vi "Read CSV File.vi"(10 "文件参数":T1={"时间列"=1, "名称行"=1, "单位行"=2, "数据首行"=3, "数据首列"=2, "分隔符"=enum."逗号"}, 11 "Path":path=path "D:/同步空间/曲线生成/原始曲线/3、增达--Data.xls") -> (2 "Data Series":T2[](array[typedef]))   [LabVIEW 2020, in "Data Viewer.lvlib"]
uses:
  Data Viewer.lvlib
  Data Serie--cluster.ctl
  File Type--enum.ctl
  <vilib>/Utility/file.llb/Read Delimited Spreadsheet (string).vi
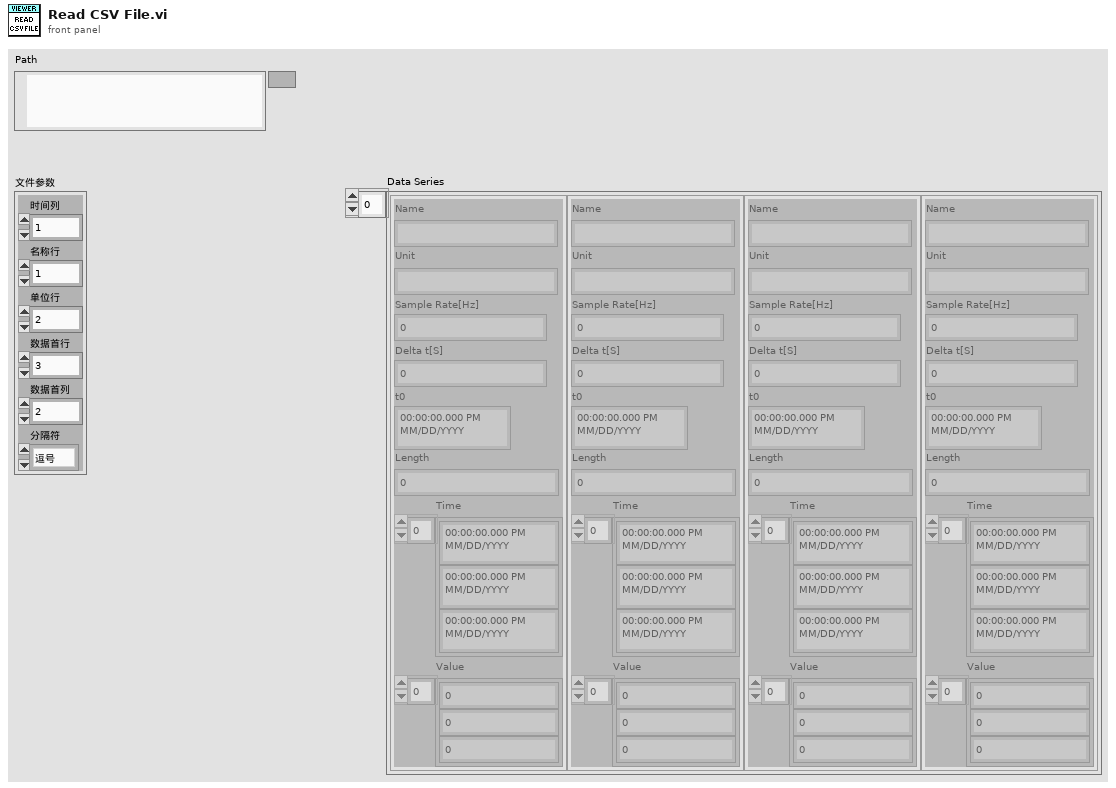
[diagram p1: front panel]
types:
  T1 = cluster{"时间列":i32, "名称行":i32, "单位行":i32, "数据首行":i32, "数据首列":i32, "分隔符":enum16{"逗号", "制表符"}}
  T2 = typedef "Data Viewer.lvlib/Data Serie--cluster.ctl" = cluster{"Name":string, "Unit":string, "Sample Rate[Hz]":dbl, "Delta t[S]":dbl, "t0":timestamp, "Length":i32, "Time":timestamp[], "Value":dbl[]}
  T3 = typedef "Data Viewer.lvlib/File Type--enum.ctl" = enum16{"伟思环境箱", "增达环境箱", "广五所环境箱", "无纸记录仪", "帕捷SA00339", "记录仪840", "记录仪8400", "记录仪MR888", "*.csv"}
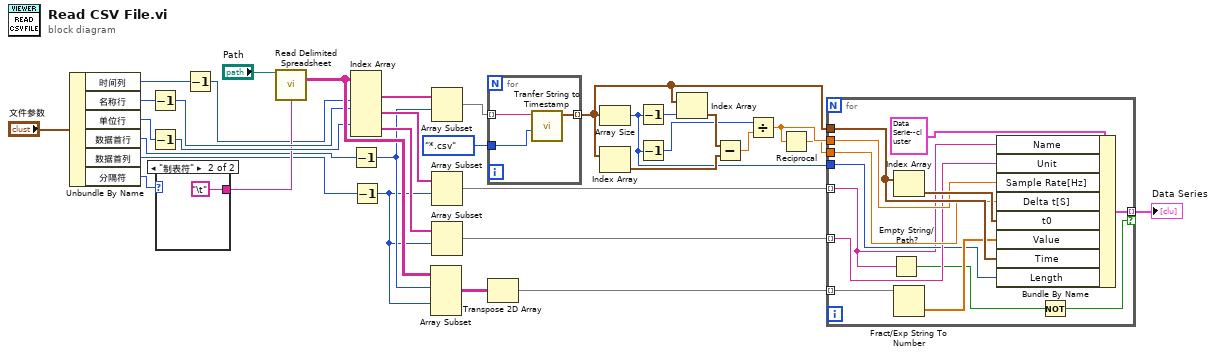
[diagram p0: block diagram]
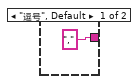
[diagram p2: hidden frame]
diagram:
  n1 = Unbundle By Name("文件参数") -> ("时间列"=w6:i32, "名称行"=w5:i32, "单位行"=w4:i32, "数据首行"=w3:i32, "数据首列"=w2:i32, "分隔符"=w1:enum16{"逗号", "制表符"})
  n2 = Decrement(x=w5) -> (x-1=w15:i32)
  n3 = Decrement(x=w4) -> (x-1=w14:i32)
  n4 = case shown="\"制表符\"" w1 {
    tunnel: ["," ("delimiter (\\t)") "\t"] -> w9
    frame "逗号", Default {
    }
    frame "制表符" {
    }
  }
  n5 = Decrement(x=w6) -> (x-1=w7:i32)
  n6 = call-poly <vilib>:"Read Delimited Spreadsheet.vi"("file path (dialog if empty)"="Path", "delimiter (\\t)"=w9) -> ("all rows"=w16:string[][])  [unwired: 8 in, 5 out]
  n7 = Index Array(array=w16, index (col) #1=w7, index (row) #2=w15, index (row) #3=w14) -> (element #1=w34:string[], element #2=w31:string[], element #3=w30:string[])  [unwired: 3 in]
  n8 = Decrement(x=w3) -> (x-1=w13:i32)
  n9 = Decrement(x=w2) -> (x-1=w12:i32)
  n10 = Array Subset(array=w16, index (row)=w13, index (col)=w12) -> (w29:string[][])  [unwired: 2 in]
  n11 = Array Subset(array=w34, index=w13) -> (w33:string[])  [unwired: 1 in]
  n12 = Array Subset(array=w31, index=w12) -> (w28:string[])  [unwired: 1 in]
  n13 = Array Subset(array=w30, index=w12) -> (w27:string[])  [unwired: 1 in]
  n14 = for {
    tunnel: w33 -> [w39] mode=indexing
    tunnel: File_Type--enum."*.csv" ("File Type") -> [w38]
    tunnel: [w37] -> w25 mode=indexing
    n15 = call "Tranfer String to Timestamp.vi"("File Type"=w38, "String"=w39) -> ("time stamp"=w37:timestamp)  [unwired: 9 in]
  }
  n16 = Transpose 2D Array(2D array=w29) -> (transposed array=w26:string[][])
  n17 = Array Size(array=w25) -> (size(s)=w10:i32)
  n18 = Index Array(array=w25) -> (element=w22:timestamp)  [unwired: 1 in]
  n19 = Decrement(x=w10) -> (x-1=w24:i32)
  n20 = Decrement(x=w10) -> (x-1=w11:i32)
  n21 = Index Array(array=w25, index=w24) -> (element=w23:timestamp)
  n22 = Subtract(x=w23, y=w22) -> (x-y=w21:dbl)
  n23 = Divide(x=w11, y=w21) -> (x/y=w20:dbl)
  n24 = Reciprocal(x=w20) -> (1/x=w19:dbl)
  n25 = for {
    tunnel: w28 -> [w42] mode=indexing
    tunnel: w27 -> [w44] mode=indexing
    tunnel: w26 -> [w49] mode=indexing
    tunnel: w25 -> [w50]
    tunnel: w20 -> [w47]
    tunnel: w19 -> [w46]
    tunnel: [w45] -> w18 mode=indexing if=w40
    tunnel: w10 -> [w43]
    n26 = Empty String/Path?(string/path=w42) -> (empty?=w41:bool)
    n27 = Index Array(array=w50) -> (element=w51:timestamp)  [unwired: 1 in]
    n28 = Fract/Exp String To Number(string=w49) -> (number=w48:dbl[])  [unwired: 3 in, 1 out]
    n29 = Bundle By Name(cluster=T2 {"Name"="", "Unit"="", "Sample Rate[Hz]"=0.0, "Delta t[S]"=0.0, "t0"=timestamp(0 s since 1904-01-01), "Length"=0, "Time"=[], "Value"=[]} ("Data Serie"), "Name"=w42, "Unit"=w44, "Sample Rate[Hz]"=w47, "Delta t[S]"=w46, "t0"=w51, "Value"=w48, "Time"=w50, "Length"=w43) -> (w45:T2)
    n30 = Not(x=w41) -> (.not. x?=w40:bool)
  }
  "Data Series" <- w18
